vi "AI_DAQ_Main.vi"() -> ()   [LabVIEW 2026]
doc: "128채널(NI 9178 x2 + NI 9203 x16) 전류 입력 측정/가시화 메인.\nUI 상태머신(Init/Wait/Update/Settings/Start/Stop/Save/Channel/Graph/Exit) + DAQ 엔진 + 그래프 팝업 루프.\n창 전체가 Picture 'Screen' 하나: 상단 버튼 6개, 128채널 타일, 하단 그래프."
panel:
  out "Screen":picture
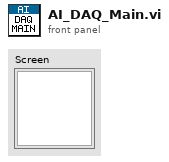
[diagram p1: front panel]
types:
  T1 = cluster{"Channels":cluster{"Name":string, "Value":dbl, "High Limit":dbl, "Low Limit":dbl, "Save":bool, "Graph":bool, "Scale Min":dbl, "Scale Max":dbl, "Unit":string}[], "Settings":cluster{"Sample Rate (Hz)":dbl, "Samples per Channel":i32, "Chassis 1 Channels":string, "Chassis 2 Channels":string, "Save Folder":path}, "Running":bool, "Logging":bool, "Data":dbl[][], "dt":dbl, "Hover":i32, "Selected":i32, "Message":string, "Log File":path}
  T2 = enum16{"Init", "Wait", "Update", "Settings", "Start", "Stop", "Save", "Channel", "Graph", "Exit"}
  T3 = cluster{"Name":string, "Value":dbl, "High Limit":dbl, "Low Limit":dbl, "Save":bool, "Graph":bool, "Scale Min":dbl, "Scale Max":dbl, "Unit":string}[]
  T4 = cluster{"Data":dbl[][], "Values":dbl[], "dt":dbl, "Running":bool, "Logging":bool, "Message":string, "Log File":path}
  T5 = cluster{"Cmd":enum16{"Start", "Stop", "Config", "Log On", "Log Off", "Exit"}, "Settings":cluster{"Sample Rate (Hz)":dbl, "Samples per Channel":i32, "Chassis 1 Channels":string, "Chassis 2 Channels":string, "Save Folder":path}, "Channels":cluster{"Name":string, "Value":dbl, "High Limit":dbl, "Low Limit":dbl, "Save":bool, "Graph":bool, "Scale Min":dbl, "Scale Max":dbl, "Unit":string}[]}
  T6 = cluster{"Left":i32, "Top":i32, "Right":i32, "Bottom":i32}
  T7 = enum16{"Start", "Stop", "Config", "Log On", "Log Off", "Exit"}
  T8 = cluster{"Sample Rate (Hz)":dbl, "Samples per Channel":i32, "Chassis 1 Channels":string, "Chassis 2 Channels":string, "Save Folder":path}
  T9 = enum16{"Init", "Wait", "Update", "Settings", "Start", "Stop", "Save", "Channel", "Graph", "Exit"}[]
  T10 = typedef "LVMouseTypeDef.ctl" = cluster{"Mouse Position":cluster{"X":i32, "Y":i32}, "Mouse Modifiers":cluster{"Button Down":bool, "Shift Mod":bool, "Menu Mod":bool, "Option Mod":bool}}
  T11 = cluster{"Rect":cluster{"left":i16, "top":i16, "right":i16, "bottom":i16}, "Fill":u32, "Fill Sel":u32, "Border":u32, "Border Sel":u32, "Text":string, "Text Color":u32, "Text Sel":u32, "Size":i16, "Bold":bool, "Group":i32, "Value":i32, "Radius":i16}[]
  T12 = cluster{"Name":string, "Value":dbl, "High Limit":dbl, "Low Limit":dbl, "Save":bool, "Graph":bool, "Scale Min":dbl, "Scale Max":dbl, "Unit":string}
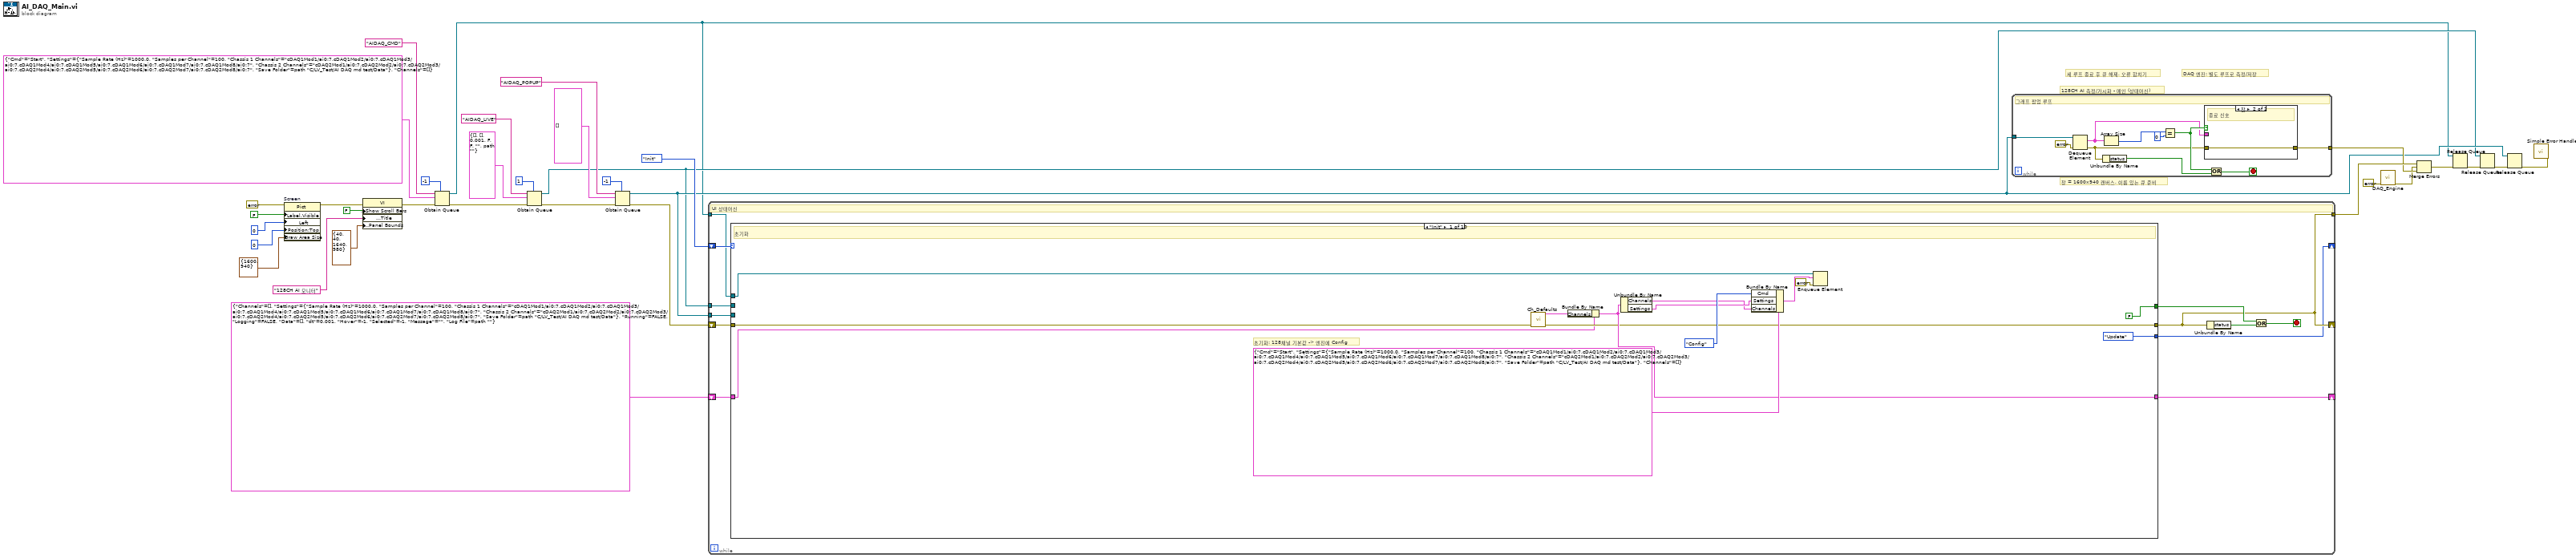
[diagram p0: block diagram]
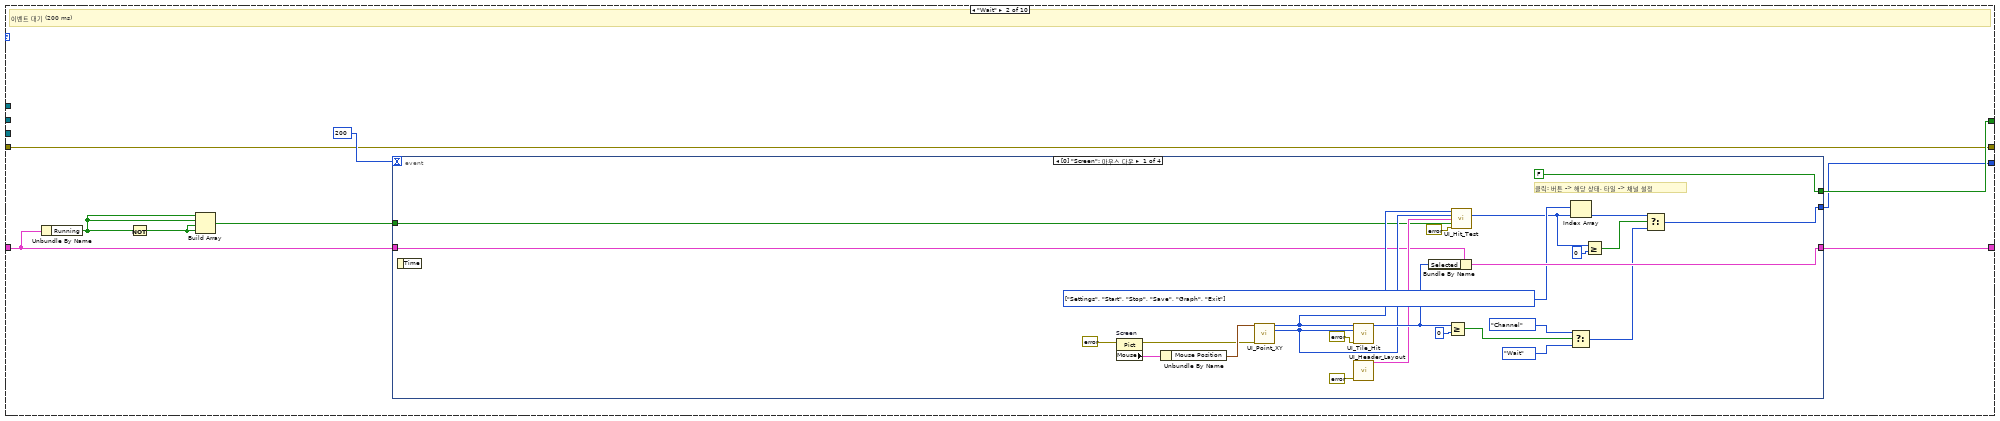
[diagram p2: hidden frame]
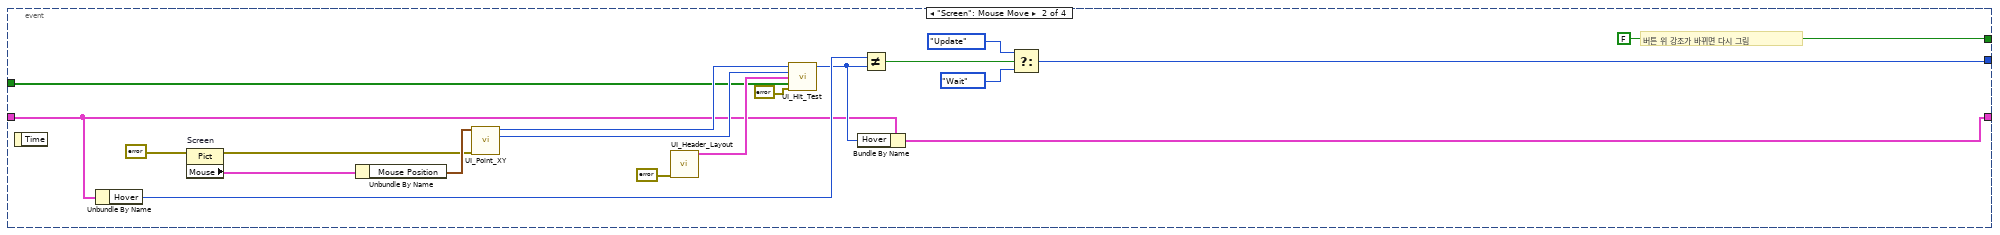
[diagram p3: hidden frame]
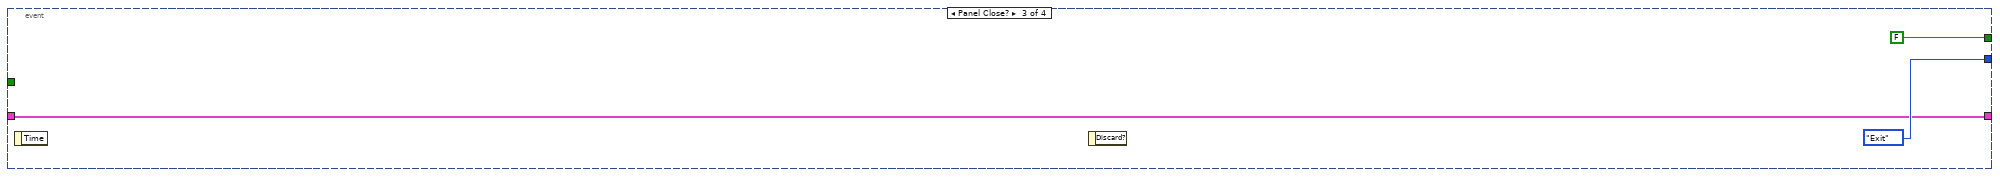
[diagram p4: hidden frame]
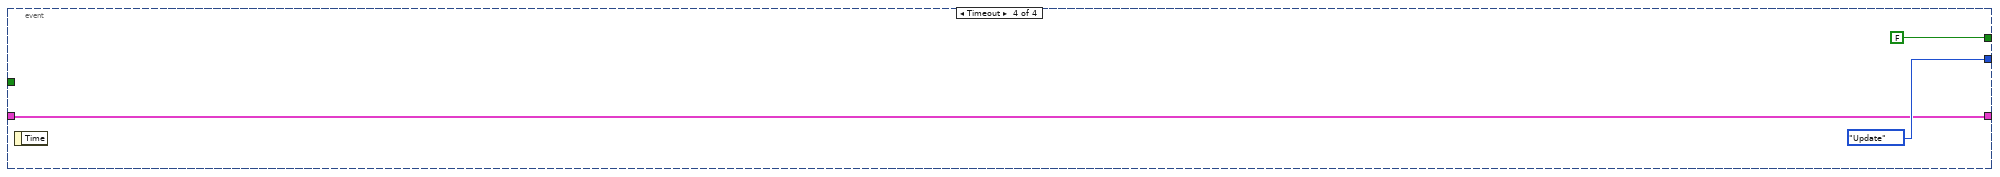
[diagram p5: hidden frame]
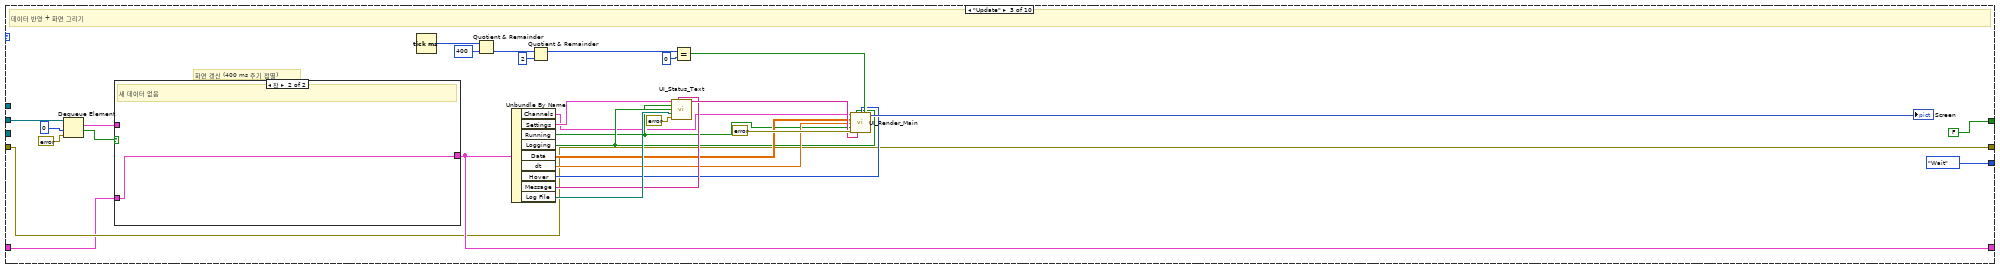
[diagram p6: hidden frame]
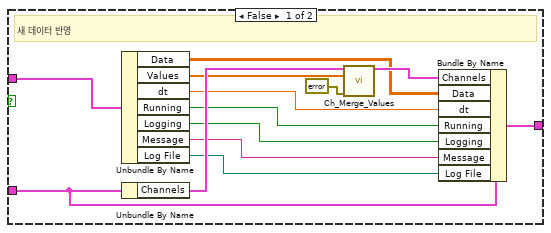
[diagram p7: hidden frame]
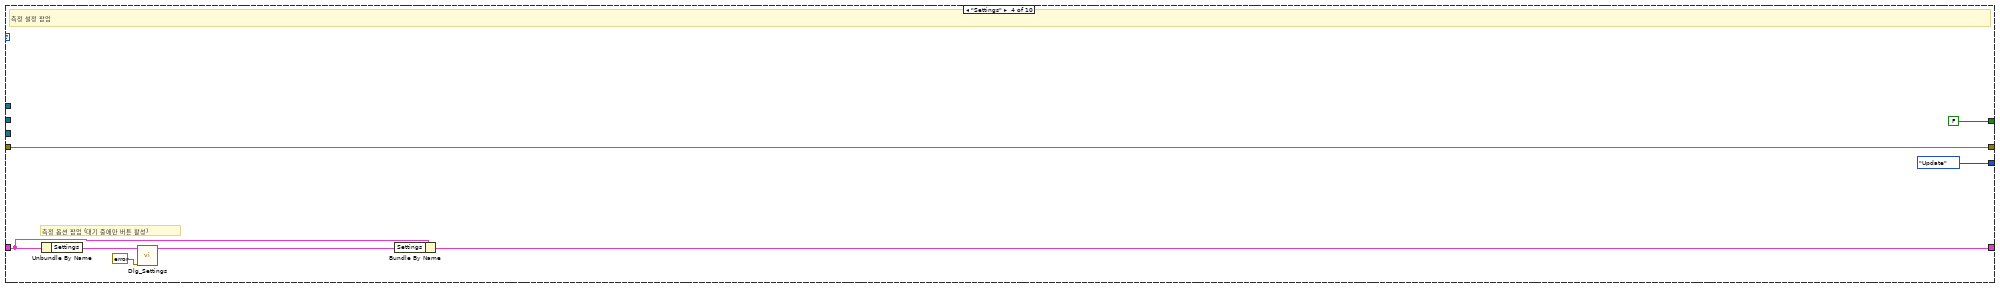
[diagram p8: hidden frame]
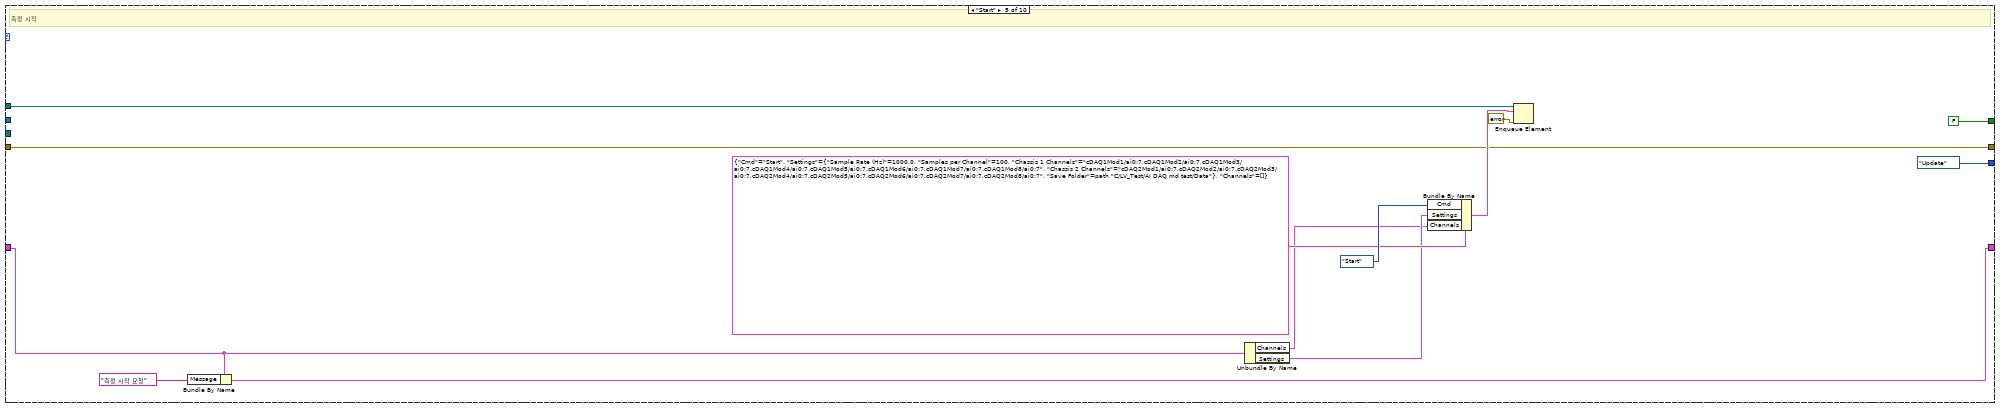
[diagram p9: hidden frame]
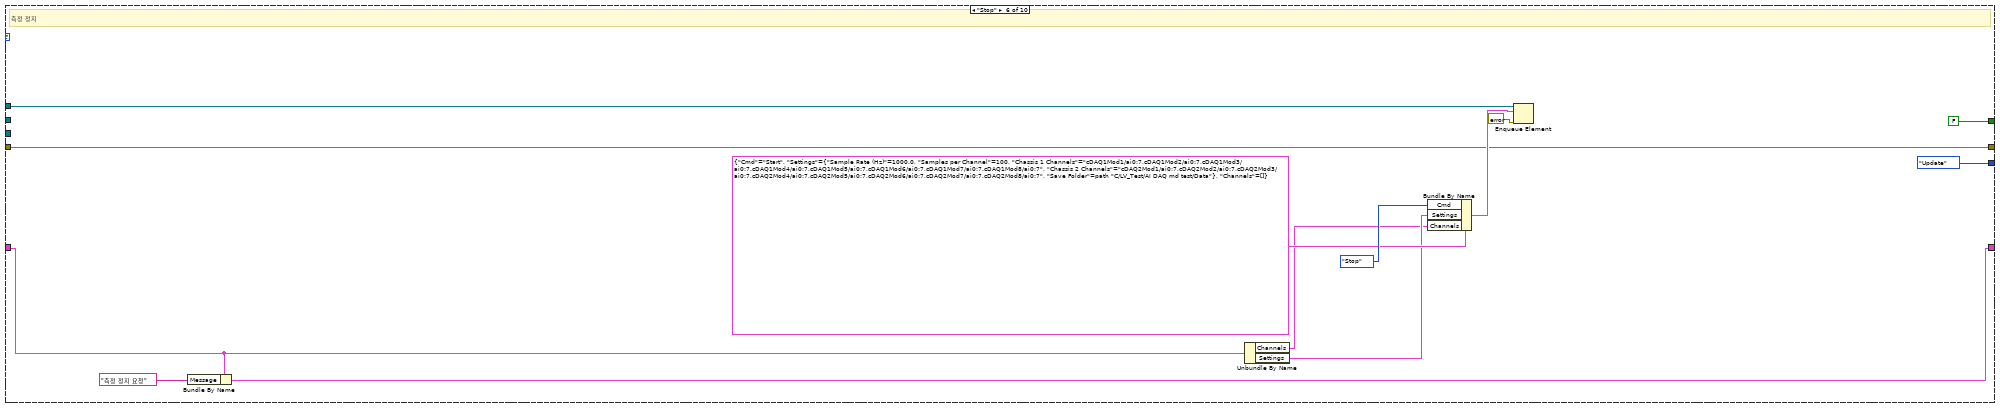
[diagram p10: hidden frame]
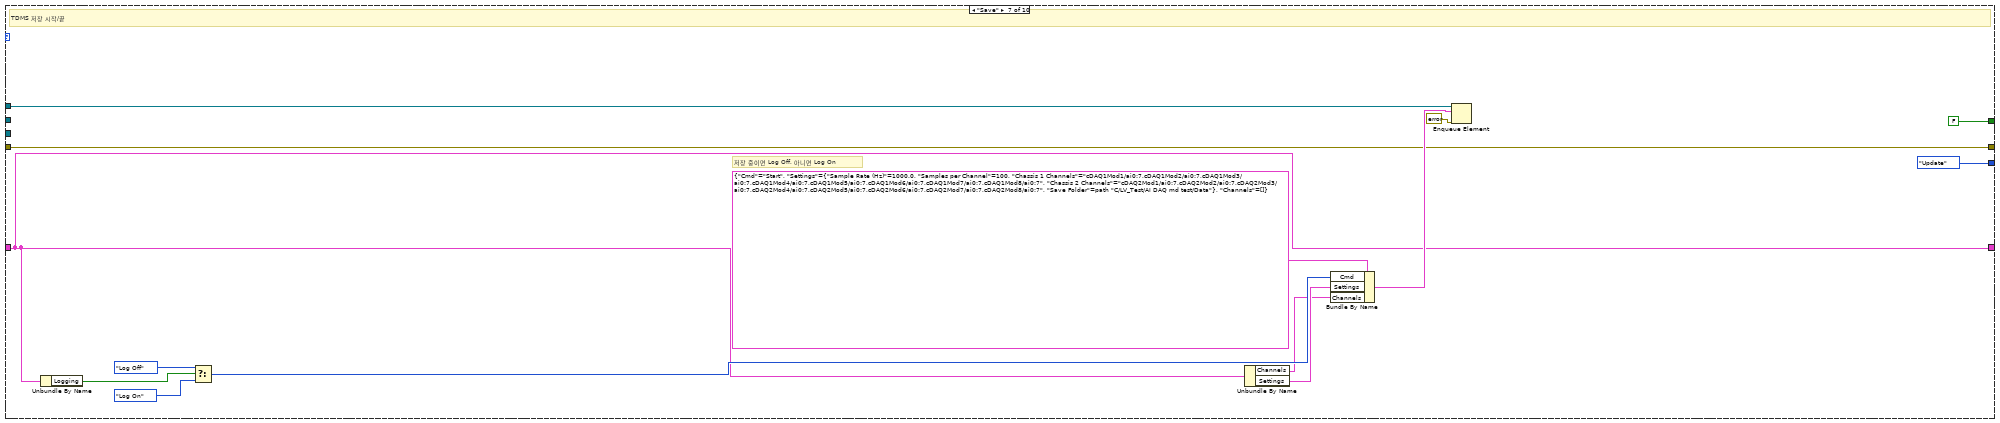
[diagram p11: hidden frame]
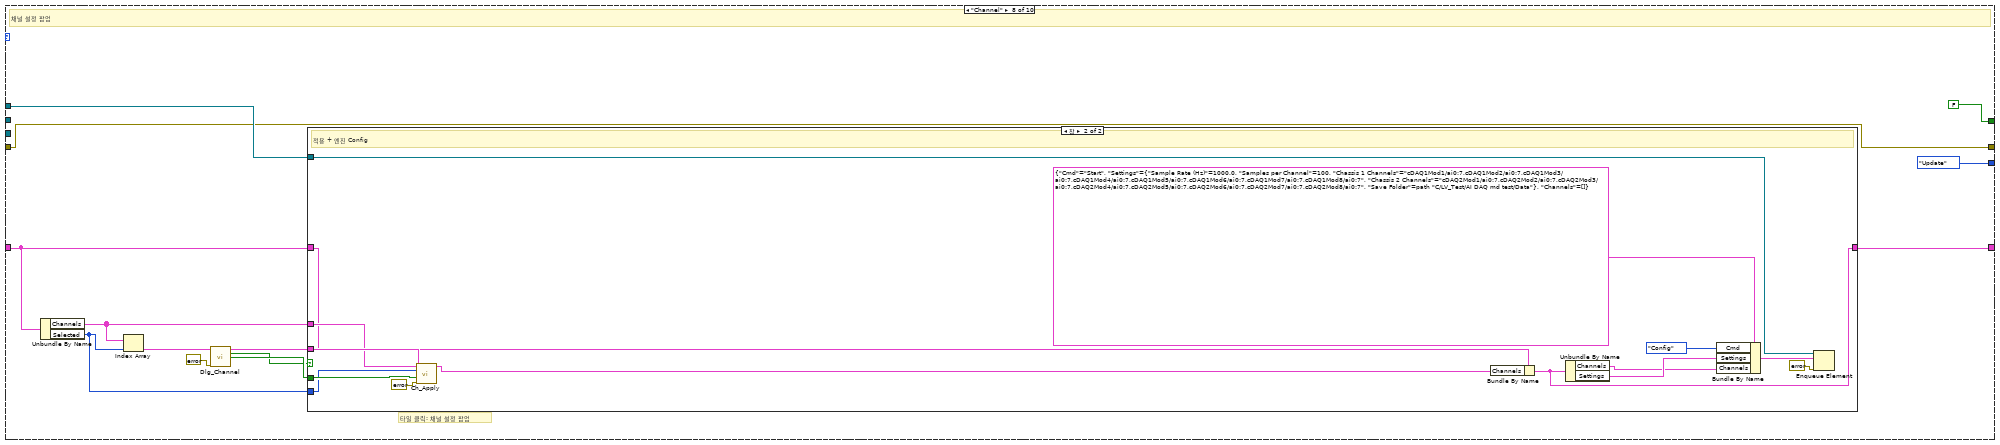
[diagram p12: hidden frame]
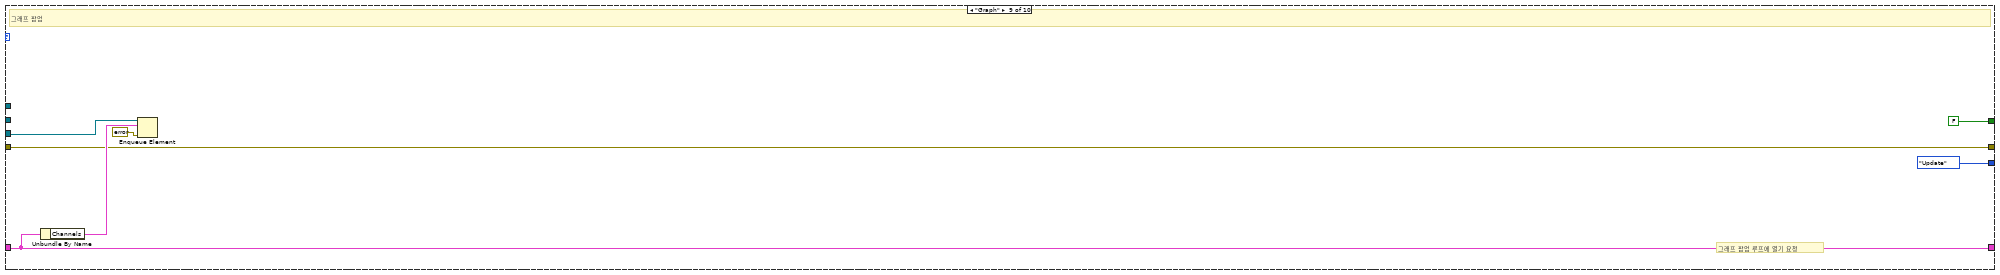
[diagram p14: hidden frame]
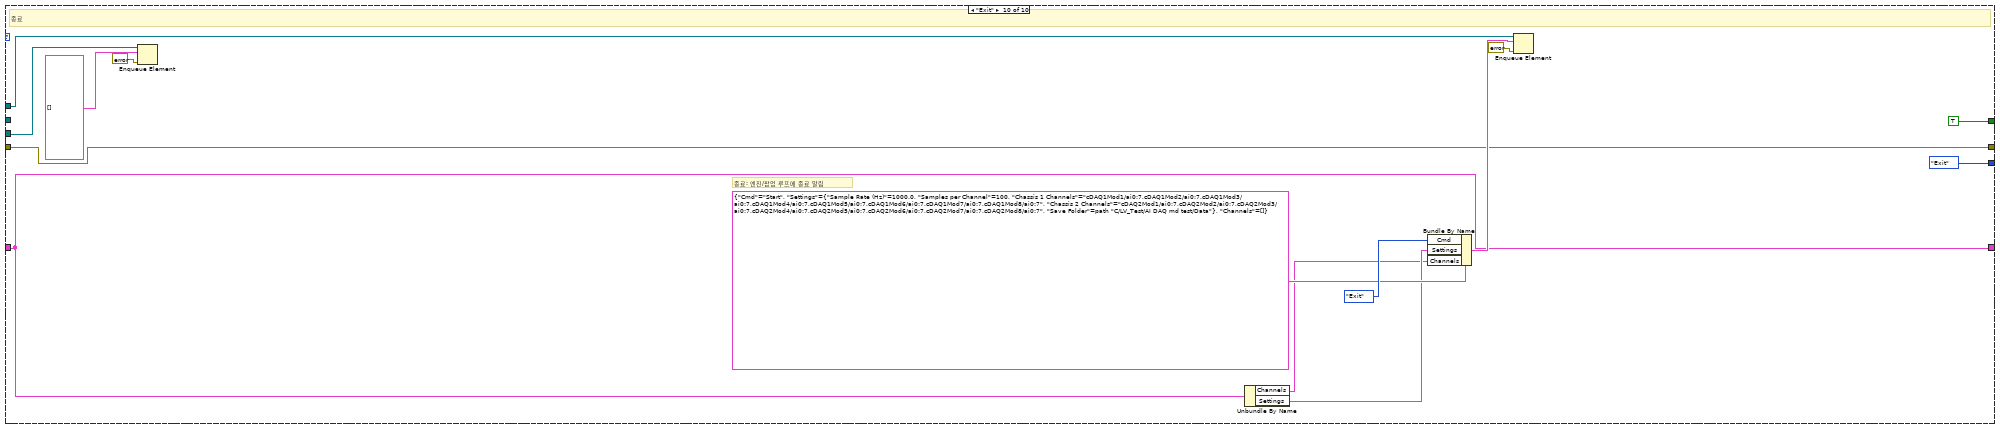
[diagram p15: hidden frame]
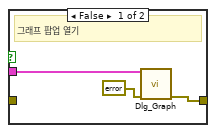
[diagram p16: hidden frame]
diagram:
  # "세 루프 종료 후 큐 해제, 오류 합치기"
  # "DAQ 엔진: 별도 루프로 측정/저장"
  # "창 = 1600x940 캔버스, 이름 있는 큐 준비"
  # "128CH AI 측정/가시화 - 메인 (상태머신)"
  n1 = property on="Screen" class="Pict"(error in=errorcluster {"status"=FALSE, "code"=0, "source"=""}, "Label.Visible"=FALSE, "Left"=0, "Position:Top"=0, "Draw Area Size"=cluster{"Width":i32, "Height":i32} {"Width"=1600, "Height"=940}) -> (error out=w6:errorcluster)  [unwired: 1 in, 1 out]
  n2 = property class="VI"(error in=w6, "Front Panel Window:Show Scroll Bars"=FALSE, "Front Panel Window:Title"="128CH AI 모니터", "Front Panel Window:Panel Bounds"=T6 {"Left"=40, "Top"=40, "Right"=1640, "Bottom"=980}) -> (error out=w10:errorcluster)  [unwired: 1 in, 1 out]
  n3 = Obtain Queue(max queue size (-1, unlimited)=-1, name (unnamed)="AIDAQ_CMD", element data type=T5 {"Cmd"=enum."Start", "Settings"={"Sample Rate (Hz)"=1000.0, "Samples per Channel"=100, "Chassis 1 Channels"="cDAQ1Mod1/ai0:7,cDAQ1Mod2/ai0:7,cDAQ1Mod3/ai0:7,cDAQ1Mod4/ai0:7,cDAQ1Mod5/ai0:7,cDAQ1Mod6/ai0:7,cDAQ1Mod7/ai0:7,cDAQ1Mod8/ai0:7", "Chassis 2 Channels"="cDAQ2Mod1/ai0:7,cDAQ2Mod2/ai0:7,cDAQ2Mod3/ai0:7,cDAQ2Mod4/ai0:7,cDAQ2Mod5/ai0:7,cDAQ2Mod6/ai0:7,cDAQ2Mod7/ai0:7,cDAQ2Mod8/ai0:7", "Save Folder"=path "C:/LV_Test/AI DAQ md test/Data"}, "Channels"=[]}, error in (no error)=w10) -> (queue out=w14:refnum<queue>, error out=w15:errorcluster)  [unwired: 1 in, 1 out]
  n4 = Obtain Queue(max queue size (-1, unlimited)=1, name (unnamed)="AIDAQ_LIVE", element data type=T4 {"Data"=[], "Values"=[], "dt"=0.001, "Running"=FALSE, "Logging"=FALSE, "Message"="", "Log File"=path ""}, error in (no error)=w15) -> (queue out=w19:refnum<queue>, error out=w20:errorcluster)  [unwired: 1 in, 1 out]
  n5 = Obtain Queue(max queue size (-1, unlimited)=-1, name (unnamed)="AIDAQ_POPUP", element data type=T3 [], error in (no error)=w20) -> (queue out=w24:refnum<queue>, error out=w25:errorcluster)  [unwired: 1 in, 1 out]
  n6 = while {
    shift-right: [w43] -> _
    shift-left: T2."Init" -> [w39]
    shift-right: [w42] -> _
    shift-left: T1 {"Channels"=[], "Settings"={"Sample Rate (Hz)"=1000.0, "Samples per Channel"=100, "Chassis 1 Channels"="cDAQ1Mod1/ai0:7,cDAQ1Mod2/ai0:7,cDAQ1Mod3/ai0:7,cDAQ1Mod4/ai0:7,cDAQ1Mod5/ai0:7,cDAQ1Mod6/ai0:7,cDAQ1Mod7/ai0:7,cDAQ1Mod8/ai0:7", "Chassis 2 Channels"="cDAQ2Mod1/ai0:7,cDAQ2Mod2/ai0:7,cDAQ2Mod3/ai0:7,cDAQ2Mod4/ai0:7,cDAQ2Mod5/ai0:7,cDAQ2Mod6/ai0:7,cDAQ2Mod7/ai0:7,cDAQ2Mod8/ai0:7", "Save Folder"=path "C:/LV_Test/AI DAQ md test/Data"}, "Running"=FALSE, "Logging"=FALSE, "Data"=[], "dt"=0.001, "Hover"=-1, "Selected"=-1, "Message"="", "Log File"=path ""} -> [w40]
    tunnel: w14 -> [w36]
    tunnel: w19 -> [w37]
    tunnel: w24 -> [w38]
    shift-right: [w44] -> _
    shift-left: w25 -> [w41]
    tunnel: [w44] -> w31
    stop <- w47 stop-if-true
    # "UI 상태머신"
    n7 = case shown="\"Init\"" w39 {
      tunnel: [T2."Update" w69 T2."Wait" T2."Update" T2."Update" T2."Update" T2."Update" T2."Update" T2."Update" T2."Exit"] -> w43
      tunnel: [FALSE w70 FALSE FALSE FALSE FALSE FALSE FALSE FALSE TRUE] -> w45
      tunnel: w40 -> [w48 w62 w122 w166 w174 w187 w200 w214 w243 w250]
      tunnel: w36 -> [w50 _ _ _ w176 w189 w202 w216 _ w252]
      tunnel: w37 -> [_ _ w124 _ _ _ _ _ _ _]
      tunnel: w41 -> [w49 w63 w123 w167 w175 w188 w201 w215 w244 w251]
      tunnel: w38 -> [_ _ _ _ _ _ _ _ w245 w253]
      tunnel: [w52 w63 w123 w167 w175 w188 w201 w215 w244 w251] -> w44
      tunnel: [w53 w68 w129 w171 w184 w197 w200 w224 w243 w250] -> w42
      frame "Init" {
        # "초기화: 128채널 기본값 -> 엔진에 Config"
        # "초기화"
        n8 = call "Ch_Defaults.vi"("error in"=w49) -> ("Channels"=w51:T3, "error out"=w52:errorcluster)  [unwired: 13 in]
        n9 = Bundle By Name(cluster=w48, "Channels"=w51) -> (w53:T1)
        n10 = Unbundle By Name(w53) -> ("Channels"=w54:T3, "Settings"=w55:T8)
        n11 = Bundle By Name(cluster=T5 {"Cmd"=enum."Start", "Settings"={"Sample Rate (Hz)"=1000.0, "Samples per Channel"=100, "Chassis 1 Channels"="cDAQ1Mod1/ai0:7,cDAQ1Mod2/ai0:7,cDAQ1Mod3/ai0:7,cDAQ1Mod4/ai0:7,cDAQ1Mod5/ai0:7,cDAQ1Mod6/ai0:7,cDAQ1Mod7/ai0:7,cDAQ1Mod8/ai0:7", "Chassis 2 Channels"="cDAQ2Mod1/ai0:7,cDAQ2Mod2/ai0:7,cDAQ2Mod3/ai0:7,cDAQ2Mod4/ai0:7,cDAQ2Mod5/ai0:7,cDAQ2Mod6/ai0:7,cDAQ2Mod7/ai0:7,cDAQ2Mod8/ai0:7", "Save Folder"=path "C:/LV_Test/AI DAQ md test/Data"}, "Channels"=[]}, "Cmd"=T7."Config", "Settings"=w55, "Channels"=w54) -> (w58:T5)
        n12 = Enqueue Element(queue=w50, element=w58, error in (no error)=errorcluster {"status"=FALSE, "code"=0, "source"=""}) -> ()  [unwired: 1 in, 3 out]
      }
      frame "Wait" {
        # "이벤트 대기 (200 ms)"
        n13 = Unbundle By Name(w62) -> ("Running"=w64:bool)
        n14 = Not(x=w64) -> (.not. x?=w65:bool)
        n15 = Build Array(w64, w64, w65, w65) -> (w66:bool[])
        n16 = event shown="[0] \"Screen\": 마우스 다운" {
          selector: _ -> [_ _ _ _]
          dyn-events: _ -> [_ _ _ _]
          timeout: 200 -> [_ _ _ _]
          tunnel: [FALSE FALSE FALSE FALSE] -> w70
          tunnel: w62 -> [w71 w97 w116 w119]
          tunnel: w66 -> [w72 w98 _ _]
          tunnel: [w95 w111 w116 w119] -> w68
          tunnel: [w94 w114 T2."Exit" T2."Update"] -> w69
          event "Screen": Mouse Down {
            w85 = T9 [enum."Settings", enum."Start", enum."Stop", enum."Save", enum."Graph", enum."Exit"] items=["Init", "Wait", "Update", "Settings", "Start", "Stop", "Save", "Channel", "Graph", "Exit"] ("Button -> State")
            # "클릭: 버튼 -> 해당 상태, 타일 -> 채널 설정"
            n17 = event-data() -> ()  [unwired: 1 in, 1 out]
            n18 = property on="Screen" class="Pict"(error in=errorcluster {"status"=FALSE, "code"=0, "source"=""}) -> (error out=w75:errorcluster, "Mouse"=w74:T10)  [unwired: 1 in, 1 out]
            n19 = Unbundle By Name(w74) -> ("Mouse Position"=w76:cluster{"X":i32, "Y":i32})
            n20 = call "UI_Point_XY.vi"("Point"=w76, "error in"=w75) -> ("X"=w77:i32, "Y"=w78:i32)  [unwired: 11 in, 1 out]
            n21 = call "UI_Tile_Hit.vi"("X"=w77, "Y"=w78, "error in"=errorcluster {"status"=FALSE, "code"=0, "source"=""}) -> ("Channel Index"=w84:i32)  [unwired: 11 in, 1 out]
            n22 = call "UI_Header_Layout.vi"("error in"=errorcluster {"status"=FALSE, "code"=0, "source"=""}) -> ("Specs"=w80:T11)  [unwired: 13 in, 1 out]
            n23 = Bundle By Name(cluster=w71, "Selected"=w84) -> (w95:T1)
            n24 = Greater Or Equal?(x=w84, y=0) -> (x >= y?=w89:bool)
            n25 = call "UI_Hit_Test.vi"("X"=w77, "Y"=w78, "Specs"=w80, "Dim Groups"=w72, "error in"=errorcluster {"status"=FALSE, "code"=0, "source"=""}) -> ("Group"=w82:i32)  [unwired: 7 in, 3 out]
            n26 = Index Array(array=w85, index=w82) -> (element=w90:T2)
            n27 = Select(t=T2."Channel", s=w89, f=T2."Wait") -> (s? t:f=w93:T2)
            n28 = Greater Or Equal?(x=w82, y=0) -> (x >= y?=w87:bool)
            n29 = Select(t=w90, s=w87, f=w93) -> (s? t:f=w94:T2)
          }
          event "Screen": Mouse Move {
            # "버튼 위 강조가 바뀌면 다시 그림"
            n30 = event-data() -> ()  [unwired: 1 in, 1 out]
            n31 = Unbundle By Name(w97) -> ("Hover"=w109:i32)
            n32 = property on="Screen" class="Pict"(error in=errorcluster {"status"=FALSE, "code"=0, "source"=""}) -> (error out=w101:errorcluster, "Mouse"=w100:T10)  [unwired: 1 in, 1 out]
            n33 = Unbundle By Name(w100) -> ("Mouse Position"=w102:cluster{"X":i32, "Y":i32})
            n34 = call "UI_Point_XY.vi"("Point"=w102, "error in"=w101) -> ("X"=w103:i32, "Y"=w104:i32)  [unwired: 11 in, 1 out]
            n35 = call "UI_Header_Layout.vi"("error in"=errorcluster {"status"=FALSE, "code"=0, "source"=""}) -> ("Specs"=w106:T11)  [unwired: 13 in, 1 out]
            n36 = call "UI_Hit_Test.vi"("X"=w103, "Y"=w104, "Specs"=w106, "Dim Groups"=w98, "error in"=errorcluster {"status"=FALSE, "code"=0, "source"=""}) -> ("Index"=w108:i32)  [unwired: 7 in, 3 out]
            n37 = Bundle By Name(cluster=w97, "Hover"=w108) -> (w111:T1)
            n38 = Not Equal?(x=w109, y=w108) -> (x != y?=w110:bool)
            n39 = Select(t=T2."Update", s=w110, f=T2."Wait") -> (s? t:f=w114:T2)
          }
          event Panel Close? {
            n40 = event-data() -> ()  [unwired: 1 in, 1 out]
            n41 = event-data() -> ()  [unwired: 2 in, 1 out]
          }
          event Timeout {
            n42 = event-data() -> ()  [unwired: 1 in, 1 out]
          }
        }
      }
      frame "Update" {
        # "화면 갱신 (400 ms 주기 점멸)"
        # "데이터 반영 + 화면 그리기"
        n43 = Dequeue Element(queue=w124, timeout in ms (-1)=0, error in (no error)=errorcluster {"status"=FALSE, "code"=0, "source"=""}) -> (element=w127:T4, timed out?=w128:bool)  [unwired: 2 out]
        n44 = case shown="참" w128 {
          tunnel: w122 -> [w152 w165]
          tunnel: w127 -> [w153 _]
          tunnel: [w164 w165] -> w129
          frame False {
            # "새 데이터 반영"
            n45 = Unbundle By Name(w153) -> ("Data"=w154:dbl[][], "Values"=w155:dbl[], "dt"=w156:dbl, "Running"=w157:bool, "Logging"=w158:bool, "Message"=w159:string, "Log File"=w160:path)
            n46 = Unbundle By Name(w152) -> ("Channels"=w161:T3)
            n47 = call "Ch_Merge_Values.vi"("Channels"=w161, "Values"=w155, "error in"=errorcluster {"status"=FALSE, "code"=0, "source"=""}) -> ("Channels out"=w163:T3)  [unwired: 11 in, 1 out]
            n48 = Bundle By Name(cluster=w152, "Channels"=w163, "Data"=w154, "dt"=w156, "Running"=w157, "Logging"=w158, "Message"=w159, "Log File"=w160) -> (w164:T1)
          }
          frame True {
            # "새 데이터 없음"
          }
        }
        n49 = Tick Count (ms)() -> (millisecond timer value=w141:u32)
        n50 = Quotient & Remainder(x=w141, y=u32 400) -> (floor(x/y)=w143:u32)  [unwired: 1 out]
        n51 = Unbundle By Name(w129) -> ("Channels"=w130:T3, "Settings"=w131:T8, "Running"=w132:bool, "Logging"=w133:bool, "Data"=w134:dbl[][], "dt"=w135:dbl, "Hover"=w136:i32, "Message"=w137:string, "Log File"=w138:path)
        n52 = Quotient & Remainder(x=w143, y=u32 2) -> (x-y*floor(x/y)=w145:u32)  [unwired: 1 out]
        n53 = call "UI_Status_Text.vi"("Settings"=w131, "Message"=w137, "Running"=w132, "Logging"=w133, "Log File"=w138, "error in"=errorcluster {"status"=FALSE, "code"=0, "source"=""}) -> ("Status"=w140:string)  [unwired: 8 in, 1 out]
        n54 = Equal?(x=w145, y=u32 0) -> (x = y?=w147:bool)
        n55 = call "UI_Render_Main.vi"("Channels"=w130, "Logging"=w133, "Hover Button"=w136, "Phase"=w147, "Data"=w134, "dt"=w135, "Running"=w132, "error in"=errorcluster {"status"=FALSE, "code"=0, "source"=""}, "Status"=w140) -> ("Picture"=→"Screen":picture)  [unwired: 5 in, 1 out]
      }
      frame "Settings" {
        # "측정 옵션 팝업 (대기 중에만 버튼 활성)"
        # "측정 설정 팝업"
        n56 = Unbundle By Name(w166) -> ("Settings"=w168:T8)
        n57 = call "Dlg_Settings.vi"("Settings"=w168, "error in"=errorcluster {"status"=FALSE, "code"=0, "source"=""}) -> ("Settings out"=w170:T8)  [unwired: 11 in, 2 out]
        n58 = Bundle By Name(cluster=w166, "Settings"=w170) -> (w171:T1)
      }
      frame "Start" {
        # "측정 시작"
        n59 = Bundle By Name(cluster=w174, "Message"="측정 시작 요청") -> (w184:T1)
        n60 = Unbundle By Name(w174) -> ("Channels"=w177:T3, "Settings"=w178:T8)
        n61 = Bundle By Name(cluster=T5 {"Cmd"=enum."Start", "Settings"={"Sample Rate (Hz)"=1000.0, "Samples per Channel"=100, "Chassis 1 Channels"="cDAQ1Mod1/ai0:7,cDAQ1Mod2/ai0:7,cDAQ1Mod3/ai0:7,cDAQ1Mod4/ai0:7,cDAQ1Mod5/ai0:7,cDAQ1Mod6/ai0:7,cDAQ1Mod7/ai0:7,cDAQ1Mod8/ai0:7", "Chassis 2 Channels"="cDAQ2Mod1/ai0:7,cDAQ2Mod2/ai0:7,cDAQ2Mod3/ai0:7,cDAQ2Mod4/ai0:7,cDAQ2Mod5/ai0:7,cDAQ2Mod6/ai0:7,cDAQ2Mod7/ai0:7,cDAQ2Mod8/ai0:7", "Save Folder"=path "C:/LV_Test/AI DAQ md test/Data"}, "Channels"=[]}, "Cmd"=T7."Start", "Settings"=w178, "Channels"=w177) -> (w181:T5)
        n62 = Enqueue Element(queue=w176, element=w181, error in (no error)=errorcluster {"status"=FALSE, "code"=0, "source"=""}) -> ()  [unwired: 1 in, 3 out]
      }
      frame "Stop" {
        # "측정 정지"
        n63 = Bundle By Name(cluster=w187, "Message"="측정 정지 요청") -> (w197:T1)
        n64 = Unbundle By Name(w187) -> ("Channels"=w190:T3, "Settings"=w191:T8)
        n65 = Bundle By Name(cluster=T5 {"Cmd"=enum."Start", "Settings"={"Sample Rate (Hz)"=1000.0, "Samples per Channel"=100, "Chassis 1 Channels"="cDAQ1Mod1/ai0:7,cDAQ1Mod2/ai0:7,cDAQ1Mod3/ai0:7,cDAQ1Mod4/ai0:7,cDAQ1Mod5/ai0:7,cDAQ1Mod6/ai0:7,cDAQ1Mod7/ai0:7,cDAQ1Mod8/ai0:7", "Chassis 2 Channels"="cDAQ2Mod1/ai0:7,cDAQ2Mod2/ai0:7,cDAQ2Mod3/ai0:7,cDAQ2Mod4/ai0:7,cDAQ2Mod5/ai0:7,cDAQ2Mod6/ai0:7,cDAQ2Mod7/ai0:7,cDAQ2Mod8/ai0:7", "Save Folder"=path "C:/LV_Test/AI DAQ md test/Data"}, "Channels"=[]}, "Cmd"=T7."Stop", "Settings"=w191, "Channels"=w190) -> (w194:T5)
        n66 = Enqueue Element(queue=w189, element=w194, error in (no error)=errorcluster {"status"=FALSE, "code"=0, "source"=""}) -> ()  [unwired: 1 in, 3 out]
      }
      frame "Save" {
        # "저장 중이면 Log Off, 아니면 Log On"
        # "TDMS 저장 시작/끝"
        n67 = Unbundle By Name(w200) -> ("Logging"=w203:bool)
        n68 = Select(t=T7."Log Off", s=w203, f=T7."Log On") -> (s? t:f=w209:T7)
        n69 = Unbundle By Name(w200) -> ("Channels"=w204:T3, "Settings"=w205:T8)
        n70 = Bundle By Name(cluster=T5 {"Cmd"=enum."Start", "Settings"={"Sample Rate (Hz)"=1000.0, "Samples per Channel"=100, "Chassis 1 Channels"="cDAQ1Mod1/ai0:7,cDAQ1Mod2/ai0:7,cDAQ1Mod3/ai0:7,cDAQ1Mod4/ai0:7,cDAQ1Mod5/ai0:7,cDAQ1Mod6/ai0:7,cDAQ1Mod7/ai0:7,cDAQ1Mod8/ai0:7", "Chassis 2 Channels"="cDAQ2Mod1/ai0:7,cDAQ2Mod2/ai0:7,cDAQ2Mod3/ai0:7,cDAQ2Mod4/ai0:7,cDAQ2Mod5/ai0:7,cDAQ2Mod6/ai0:7,cDAQ2Mod7/ai0:7,cDAQ2Mod8/ai0:7", "Save Folder"=path "C:/LV_Test/AI DAQ md test/Data"}, "Channels"=[]}, "Cmd"=w209, "Settings"=w205, "Channels"=w204) -> (w210:T5)
        n71 = Enqueue Element(queue=w202, element=w210, error in (no error)=errorcluster {"status"=FALSE, "code"=0, "source"=""}) -> ()  [unwired: 1 in, 3 out]
      }
      frame "Channel" {
        # "타일 클릭: 채널 설정 팝업"
        # "채널 설정 팝업"
        n72 = Unbundle By Name(w214) -> ("Channels"=w217:T3, "Selected"=w218:i32)
        n73 = Index Array(array=w217, index=w218) -> (element=w219:T12)
        n74 = call "Dlg_Channel.vi"("Channel"=w219, "error in"=errorcluster {"status"=FALSE, "code"=0, "source"=""}) -> ("Channel out"=w221:T12, "OK?"=w222:bool, "Apply All"=w223:bool)  [unwired: 10 in, 1 out]
        n75 = case shown="참" w222 {
          tunnel: w214 -> [w227 w228]
          tunnel: w217 -> [_ w229]
          tunnel: w218 -> [_ w230]
          tunnel: w221 -> [_ w231]
          tunnel: w223 -> [_ w232]
          tunnel: w216 -> [_ w233]
          tunnel: [w227 w236] -> w224
          frame False {
            # "취소"
          }
          frame True {
            # "적용 + 엔진 Config"
            n76 = call "Ch_Apply.vi"("Channels"=w229, "Index"=w230, "Channel"=w231, "Apply All"=w232, "error in"=errorcluster {"status"=FALSE, "code"=0, "source"=""}) -> ("Channels out"=w235:T3)  [unwired: 9 in, 1 out]
            n77 = Bundle By Name(cluster=w228, "Channels"=w235) -> (w236:T1)
            n78 = Unbundle By Name(w236) -> ("Channels"=w237:T3, "Settings"=w238:T8)
            n79 = Bundle By Name(cluster=T5 {"Cmd"=enum."Start", "Settings"={"Sample Rate (Hz)"=1000.0, "Samples per Channel"=100, "Chassis 1 Channels"="cDAQ1Mod1/ai0:7,cDAQ1Mod2/ai0:7,cDAQ1Mod3/ai0:7,cDAQ1Mod4/ai0:7,cDAQ1Mod5/ai0:7,cDAQ1Mod6/ai0:7,cDAQ1Mod7/ai0:7,cDAQ1Mod8/ai0:7", "Chassis 2 Channels"="cDAQ2Mod1/ai0:7,cDAQ2Mod2/ai0:7,cDAQ2Mod3/ai0:7,cDAQ2Mod4/ai0:7,cDAQ2Mod5/ai0:7,cDAQ2Mod6/ai0:7,cDAQ2Mod7/ai0:7,cDAQ2Mod8/ai0:7", "Save Folder"=path "C:/LV_Test/AI DAQ md test/Data"}, "Channels"=[]}, "Cmd"=T7."Config", "Settings"=w238, "Channels"=w237) -> (w241:T5)
            n80 = Enqueue Element(queue=w233, element=w241, error in (no error)=errorcluster {"status"=FALSE, "code"=0, "source"=""}) -> ()  [unwired: 1 in, 3 out]
          }
        }
      }
      frame "Graph" {
        # "그래프 팝업 루프에 열기 요청"
        # "그래프 팝업"
        n81 = Unbundle By Name(w243) -> ("Channels"=w246:T3)
        n82 = Enqueue Element(queue=w245, element=w246, error in (no error)=errorcluster {"status"=FALSE, "code"=0, "source"=""}) -> ()  [unwired: 1 in, 3 out]
      }
      frame "Exit" {
        # "종료: 엔진/팝업 루프에 종료 알림"
        # "종료"
        n83 = Enqueue Element(queue=w253, element=T3 [], error in (no error)=errorcluster {"status"=FALSE, "code"=0, "source"=""}) -> ()  [unwired: 1 in, 3 out]
        n84 = Unbundle By Name(w250) -> ("Channels"=w254:T3, "Settings"=w255:T8)
        n85 = Bundle By Name(cluster=T5 {"Cmd"=enum."Start", "Settings"={"Sample Rate (Hz)"=1000.0, "Samples per Channel"=100, "Chassis 1 Channels"="cDAQ1Mod1/ai0:7,cDAQ1Mod2/ai0:7,cDAQ1Mod3/ai0:7,cDAQ1Mod4/ai0:7,cDAQ1Mod5/ai0:7,cDAQ1Mod6/ai0:7,cDAQ1Mod7/ai0:7,cDAQ1Mod8/ai0:7", "Chassis 2 Channels"="cDAQ2Mod1/ai0:7,cDAQ2Mod2/ai0:7,cDAQ2Mod3/ai0:7,cDAQ2Mod4/ai0:7,cDAQ2Mod5/ai0:7,cDAQ2Mod6/ai0:7,cDAQ2Mod7/ai0:7,cDAQ2Mod8/ai0:7", "Save Folder"=path "C:/LV_Test/AI DAQ md test/Data"}, "Channels"=[]}, "Cmd"=T7."Exit", "Settings"=w255, "Channels"=w254) -> (w258:T5)
        n86 = Enqueue Element(queue=w252, element=w258, error in (no error)=errorcluster {"status"=FALSE, "code"=0, "source"=""}) -> ()  [unwired: 1 in, 3 out]
      }
    }
    n87 = Unbundle By Name(w44) -> ("status"=w46:bool)
    n88 = Or(x=w45, y=w46) -> (x .or. y?=w47:bool)
  }
  n89 = while {
    tunnel: w24 -> [w264]
    tunnel: [w271] -> w28
    stop <- w273 stop-if-true
    # "그래프 팝업 루프"
    n90 = Dequeue Element(queue=w264, error in (no error)=errorcluster {"status"=FALSE, "code"=0, "source"=""}) -> (element=w266:T3, error out=w267:errorcluster)  [unwired: 1 in, 2 out]
    n91 = Unbundle By Name(w267) -> ("status"=w272:bool)
    n92 = Array Size(array=w266) -> (size(s)=w268:i32)
    n93 = Equal?(x=w268, y=0) -> (x = y?=w270:bool)
    n94 = case shown="참" w270 {
      tunnel: w266 -> [w274 _]
      tunnel: w267 -> [_ w277]
      tunnel: [w276 w277] -> w271
      frame False {
        # "그래프 팝업 열기"
        n95 = call "Dlg_Graph.vi"("Channels"=w274, "error in"=errorcluster {"status"=FALSE, "code"=0, "source"=""}) -> ("error out"=w276:errorcluster)  [unwired: 13 in]
      }
      frame True {
        # "종료 신호"
      }
    }
    n96 = Or(x=w270, y=w272) -> (x .or. y?=w273:bool)
  }
  n97 = call "DAQ_Engine.vi"("error in"=errorcluster {"status"=FALSE, "code"=0, "source"=""}) -> ("error out"=w27:errorcluster)  [unwired: 14 in]
  n98 = Merge Errors(w31, w27, w28) -> (w32:errorcluster)
  n99 = Release Queue(queue=w14, error in (no error)=w32) -> (error out=w33:errorcluster)  [unwired: 1 in, 2 out]
  n100 = Release Queue(queue=w19, error in (no error)=w33) -> (error out=w34:errorcluster)  [unwired: 1 in, 2 out]
  n101 = Release Queue(queue=w24, error in (no error)=w34) -> (error out=w35:errorcluster)  [unwired: 1 in, 2 out]
  n102 = call <vilib>:"Simple Error Handler.vi"("error in (no error)"=w35) -> ()  [unwired: 4 in, 5 out]
